vi "Sample.vi"(8 "错误输入（无错误）":errorcluster, 10 "VISA资源名称":refnum<visa-resource-name>) -> (0 "error out":errorcluster, 2 "Data Out":dbl[](array[numeric]) format="%.2f")   [LabVIEW 2026, in "UI-距离测量.lvlib" / "Acquisition.lvlib"]
uses:
  Acquisition.lvlib
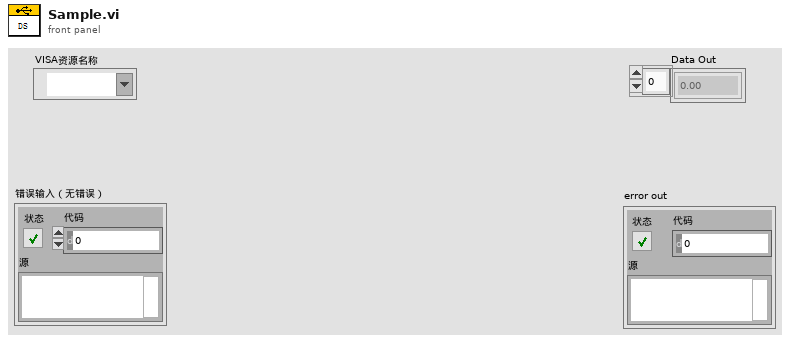
[diagram p1: front panel]
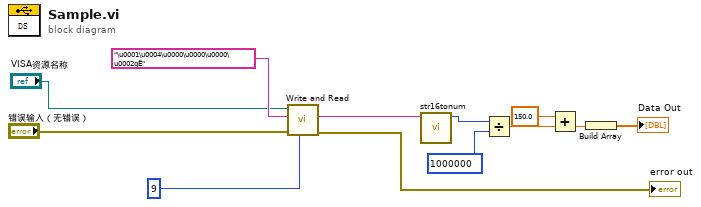
[diagram p0: block diagram]
diagram:
  n1 = call "Write and Read.vi"("读取字节数"=u32 9, "错误输入（无错误）"="错误输入（无错误）", "Command"="\u0001\u0004\u0000\u0000\u0000\u0002qË", "VISA输入"="VISA资源名称") -> ("错误输出"=→"error out":errorcluster, "read buffer"=w2:string)  [unwired: 5 in, 1 out]
  n2 = call "str16tonum.vi"("字符串"=w2) -> ("数值"=w5:i32)  [unwired: 10 in]
  n3 = Divide(x=w5, y=1000000) -> (x/y=w7:dbl)
  n4 = Add(x=150.0, y=w7) -> (x+y=w4:dbl)
  n5 = Build Array(w4) -> (→"Data Out":dbl[])
